vi "MW_Duration_Adjustment.vi"(10 "Numeric":i32) -> ()   [LabVIEW 2024]
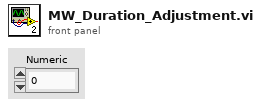
[diagram p1: front panel]
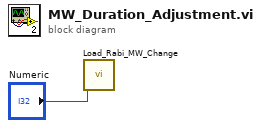
[diagram p0: block diagram]
diagram:
  n1 = call "Load_Rabi_MW_Change.vi"("Numeric"="Numeric") -> ()  [unwired: 11 in]
